vi "evo irimager trigger shutter flag.vi"() -> (3 "function return":i32)   [LabVIEW 2025, in "libirimager_direct_binding.lvlib"]
doc: "DIRECT_API int evo_irimager_trigger_shutter_flag();"
uses:
  libirimager_direct_binding.lvlib
  libirimager.dll
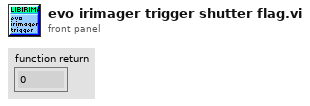
[diagram p1: front panel]
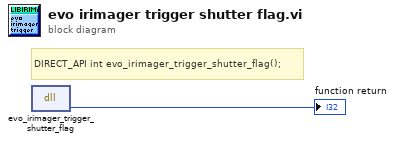
[diagram p0: block diagram]
diagram:
  # "DIRECT_API int evo_irimager_trigger_shutter_flag();"
  n1 = dll-call lib="C:/Users/mayhe/OneDrive/Documents/GitHub/In-situ-monitoring-of-powder-bed-fusion-additive-manufacturing/system_development/Orichalcum/v0.2/Software_design/thermal-camera/VI/labview/libirimager.dll" fn="evo_irimager_trigger_shutter_flag"() -> ("Rückgabetyp"=→"function return":i32)  [unwired: 3 in, 2 out]
